vi "ReferenceResolver.vi"(8 "error In":errorcluster, 11 "vi path":string) -> (0 "error out":errorcluster, 1 "VI out":refnum<vi>, 2 "UseGobject":bool, 3 "GObject":refnum<vi>, 5 "path":path)   [LabVIEW 2020]
uses:
  <vilib>/Utility/traverseref.llb/TRef TravTarget.ctl
  <vilib>/Utility/traverseref.llb/VI Scripting - Traverse.lvlib
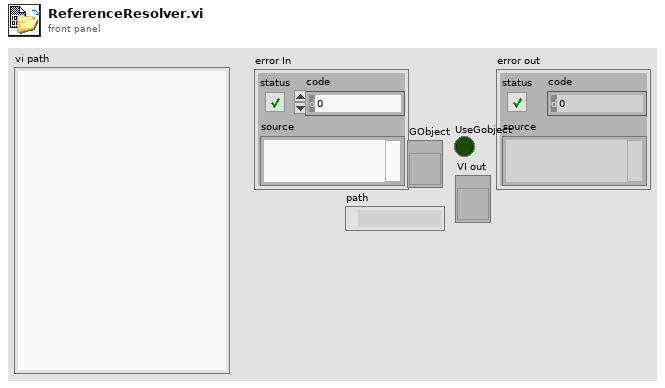
[diagram p1: front panel]
types:
  T1 = typedef "TRef TravTarget.ctl" = enum16{"FP", "BD", "Other"}
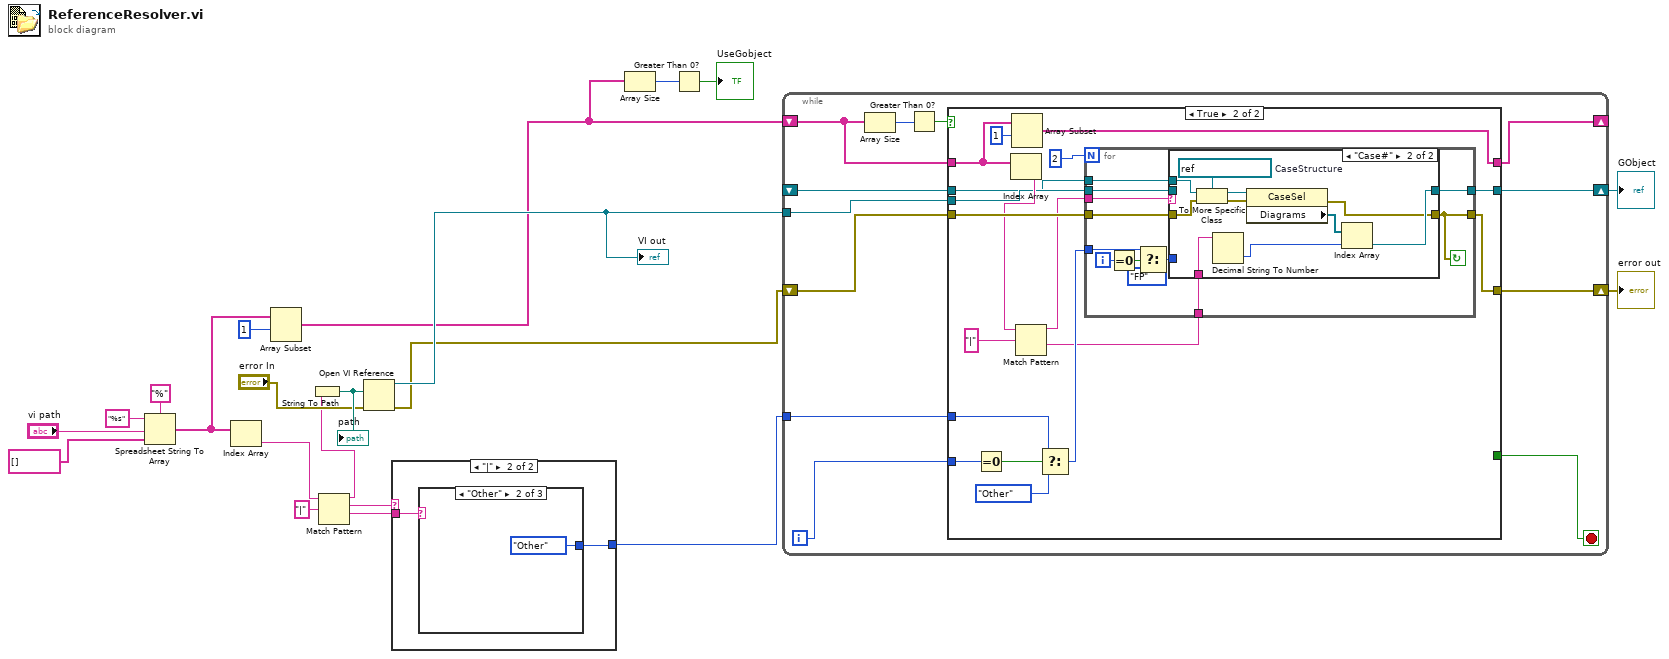
[diagram p0: block diagram]
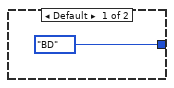
[diagram p2: hidden frame]
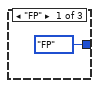
[diagram p3: hidden frame]
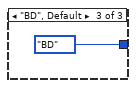
[diagram p4: hidden frame]
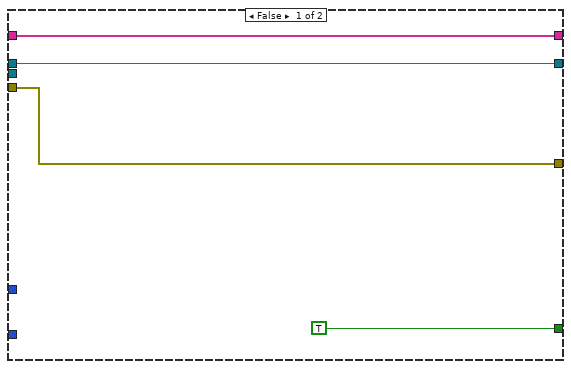
[diagram p5: hidden frame]
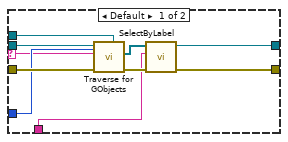
[diagram p6: hidden frame]
diagram:
  n1 = Spreadsheet String To Array(delimiter (Tab)="%", format string="%s", spreadsheet string="vi path", array type (2D Dbl)=string[] []) -> (array=w13:string[])
  n2 = Index Array(array=w13) -> (element=w6:string)  [unwired: 1 in]
  n3 = Array Subset(array=w13, index=1) -> (w8:string[])  [unwired: 1 in]
  n4 = Match Pattern(string=w6, regular expression="|") -> (before substring=w4:string, match substring=w3:string, after substring=w2:string)  [unwired: 1 in, 1 out]
  n5 = String To Path(string=w4) -> (path=w17:path)
  "path" <- w17
  n6 = Open VI Reference(vi path=w17, error in (no error)="error In") -> (vi reference=w11:refnum<vi>, error out=w10:errorcluster)  [unwired: 4 in]
  "VI out" <- w11
  n7 = case shown="\"|\"" w3 {
    tunnel: w2 -> [_ w24]
    tunnel: [TRef_TravTarget."BD" ("Traverse Target") w23] -> w1
    frame Default {
    }
    frame "|" {
      n8 = case shown="\"Other\"" w24 {
        tunnel: [TRef_TravTarget."FP" ("Traverse Target") TRef_TravTarget."Other" ("Traverse Target") TRef_TravTarget."BD" ("Traverse Target")] -> w23
        frame "FP" {
        }
        frame "Other" {
        }
        frame "BD", Default {
        }
      }
    }
  }
  n9 = Array Size(array=w8) -> (size(s)=w19:i32)
  n10 = Greater Than 0?(x=w19) -> (x > 0?=→"UseGobject":bool)
  n11 = while {
    shift-right: [w30] -> w21
    shift-left: _ -> [w37]
    shift-right: [w34] -> _
    shift-left: w8 -> [w36]
    shift-right: [w29] -> w20
    shift-left: w10 -> [w33]
    tunnel: w11 -> [w31]
    tunnel: w1 -> [w28]
    i -> [w32]
    stop <- w35 stop-if-true
    n12 = Array Size(array=w36) -> (size(s)=w39:i32)
    n13 = Greater Than 0?(x=w39) -> (x > 0?=w38:bool)
    n14 = case shown="True" w38 {
      tunnel: w37 -> [w41 w51]
      tunnel: [w41 w54] -> w30
      tunnel: w36 -> [w42 w60]
      tunnel: [TRUE _] -> w35
      tunnel: [w42 w58] -> w34
      tunnel: w33 -> [w40 w61]
      tunnel: w32 -> [_ w53]
      tunnel: w31 -> [_ w52]
      tunnel: [w40 w47] -> w29
      tunnel: w28 -> [_ w44]
      frame False {
      }
      frame True {
        n15 = Equal To 0?(x=w53) -> (x = 0?=w50:bool)
        n16 = Index Array(array=w60) -> (element=w56:string)  [unwired: 1 in]
        n17 = Array Subset(array=w60, index=1) -> (w58:string[])  [unwired: 1 in]
        n18 = Match Pattern(string=w56, regular expression="|") -> (before substring=w55:string, after substring=w46:string)  [unwired: 1 in, 2 out]
        n19 = Select(t=w44, s=w50, f=TRef_TravTarget."Other") -> (s? t:f=w48:T1)
        n20 = for {
          N: 2 -> [_]
          tunnel: w55 -> [w62]
          tunnel: [w72] -> w54
          tunnel: w52 -> [w71]
          tunnel: w51 -> [w70]
          tunnel: w48 -> [w65]
          tunnel: w46 -> [w69]
          tunnel: w61 -> [w73]
          tunnel: [w68] -> w47
          i -> [w67]
          stop <- w68 continue-if-true
          n21 = Equal To 0?(x=w67) -> (x = 0?=w66:bool)
          n22 = Select(t=w65, s=w66, f=TRef_TravTarget."FP") -> (s? t:f=w63:T1)
          n23 = case shown="\"Case#\"" w62 {
            selector: w62 -> [w74 _]
            tunnel: w73 -> [w83 w93]
            tunnel: [w81 w85] -> w72
            tunnel: w71 -> [w80 _]
            tunnel: w70 -> [w79 w92]
            tunnel: w69 -> [w77 w90]
            tunnel: [w76 w84] -> w68
            tunnel: w63 -> [w75 _]
            frame Default {
              n24 = call <vilib>:"Traverse for GObjects.vi"("Other Refnum"=w79, "Traverse Target"=w75, "error in (no error)"=w83, "Class Name"=w74, "VI Refnum"=w80) -> ("error out"=w82:errorcluster, "References"=w78:refnum<vi>[])  [unwired: 3 in, 2 out]
              n25 = call "SelectByLabel.vi"("error in (no error)"=w82, "String"=w77, "References"=w78) -> ("error out"=w76:errorcluster, "GObject out"=w81:refnum<vi>)  [unwired: 7 in]
            }
            frame "Case#" {
              w91 = refnum<vi> refnum  # CaseStructure
              n26 = To More Specific Class(target class=w91, reference=w92, error in=w93) -> (specific class reference=w89:refnum<vi>, error out=w88:errorcluster)
              n27 = Decimal String To Number(string=w90) -> (number=w86:i32)  [unwired: 2 in, 1 out]
              n28 = property class="CaseSel"(reference=w89, error in=w88) -> (error out=w84:errorcluster, "Diagrams"=w87:refnum<vi>[])  [unwired: 1 out]
              n29 = Index Array(array=w87, index=w86) -> (element=w85:refnum<vi>)
            }
          }
        }
      }
    }
  }
  "GObject" <- w21
  "error out" <- w20
